vi "Prompt User for Init Type.vi"(8 "error in (no error)":errorcluster) -> (0 "error out":errorcluster, 2 "Group? out":bool, 3 "Path out":path)   [LabVIEW 2019, in "FPGA Addon System Explorer.lvlib"]
uses:
  FPGA Addon System Explorer.lvlib
panel:
  in  "Group?":bool
  in  "New Instance?":bool
  in  "OK":bool
  in  "Path":path
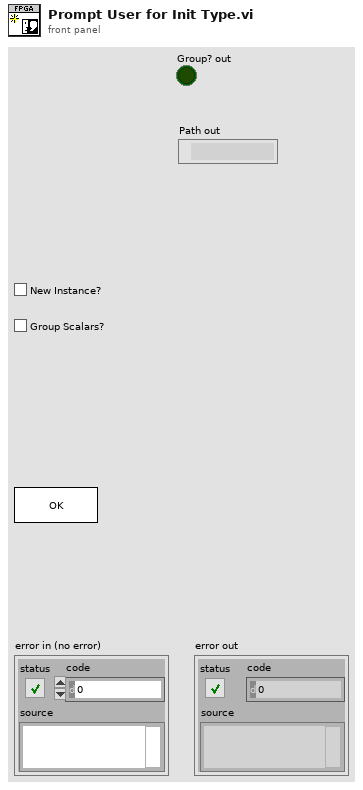
[diagram p1: front panel]
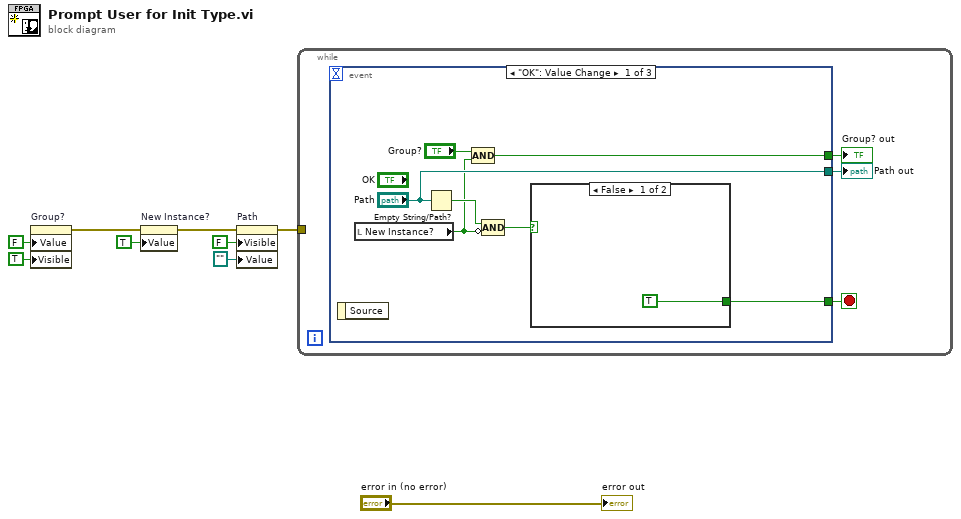
[diagram p0: block diagram]
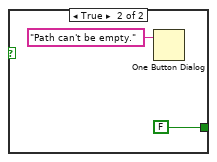
[diagram p2: hidden frame]
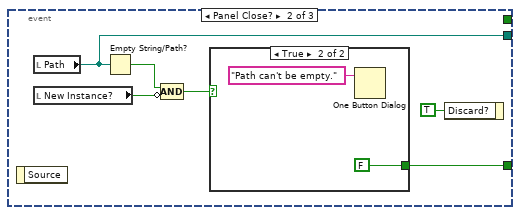
[diagram p3: hidden frame]
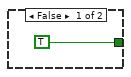
[diagram p4: hidden frame]
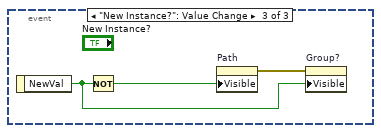
[diagram p5: hidden frame]
diagram:
  n1 = property on="Group?" class="Bool (strict)"("Value"=FALSE ("Group?"), "Visible"=TRUE) -> (error out=w2:errorcluster)  [unwired: 2 in, 1 out]
  n2 = property on="New Instance?" class="Bool (strict)"(error in=w2, "Value"=TRUE ("New Instance?")) -> (error out=w6:errorcluster)  [unwired: 1 in, 1 out]
  n3 = property on="Path" class="Path"(error in=w6, "Visible"=FALSE, "Value"=path "") -> (error out=w8:errorcluster)  [unwired: 1 in, 1 out]
  n4 = while {
    tunnel: w8 -> [_]
    stop <- w12 stop-if-true
    n5 = event shown="[0] \"OK\": Value Change" {
      selector: _ -> [_ _ _]
      dyn-events: _ -> [_ _ _]
      timeout: _ -> [_ _ _]
      tunnel: [w19 w28 _] -> w12
      tunnel: ["Path" w23 _] -> w11
      tunnel: [w14 _ _] -> w10
      event "OK": Value Change {
        n6 = event-data() -> ()  [unwired: 1 in, 1 out]
        n7 = local read "New Instance?"() -> (w13:bool)
        n8 = Empty String/Path?(string/path="Path") -> (empty?=w17:bool)
        n9 = Compound Arithmetic op=AND("Group?", w13) -> (w14:bool)
        n10 = Compound Arithmetic op=AND(w17, invert w13) -> (w16:bool)
        n11 = case shown="False" w16 {
          tunnel: [TRUE FALSE] -> w19
          frame False {
          }
          frame True {
            n12 = One Button Dialog(message="Path can't be empty.") -> ()  [unwired: 1 in, 1 out]
          }
        }
      }
      event Panel Close? {
        n13 = event-data() -> ()  [unwired: 1 in, 1 out]
        n14 = local read "Path"() -> (w23:path)
        n15 = local read "New Instance?"() -> (w27:bool)
        n16 = Empty String/Path?(string/path=w23) -> (empty?=w26:bool)
        n17 = Compound Arithmetic op=AND(w26, invert w27) -> (w25:bool)
        n18 = case shown="True" w25 {
          tunnel: [TRUE FALSE] -> w28
          frame False {
          }
          frame True {
            n19 = One Button Dialog(message="Path can't be empty.") -> ()  [unwired: 1 in, 1 out]
          }
        }
        n20 = event-data("Discard?"=TRUE) -> ()  [unwired: 1 in, 1 out]
      }
      event "New Instance?": Value Change {
        n21 = event-data() -> ("NewVal"=w32:bool)  [unwired: 1 in]
        n22 = Not(x=w32) -> (.not. x?=w34:bool)
        n23 = property on="Path" class="Path"("Visible"=w34) -> (error out=w33:errorcluster)  [unwired: 2 in, 1 out]
        n24 = property on="Group?" class="Bool (strict)"(error in=w33, "Visible"=w32) -> ()  [unwired: 1 in, 2 out]
      }
    }
    "Path out" <- w11
    "Group? out" <- w10
  }
  "error out" <- "error in (no error)"
